vi "RUN regulateur MODBUS EPC3000.vi"(2 "Commentaires":string, 3 "Fichier rapport":path) -> (0 "error out":errorcluster caption="entrée d'erreur (pas d'erreur)", 1 "annulé":bool)   [LabVIEW 2022 SP3]
uses:
  Enum/Enum r5.ctl
  Variables globales/Variables glob EUROTHERM.vi
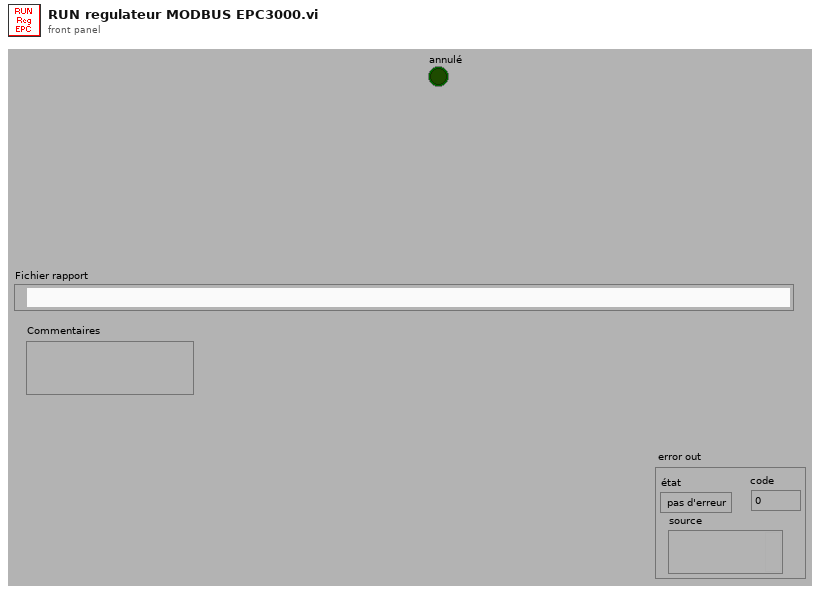
[diagram p1: front panel]
types:
  T1 = typedef "Enum r5.ctl" = enum16{"déja en run", "mesure hors gamme", "fichier rapport", "envoi run", "fin"}
  T2 = cluster{"Noms voies select acqui 1COM":string[]}[]
  T3 = typedef "Semaphore RefNum" = refnum<k1>
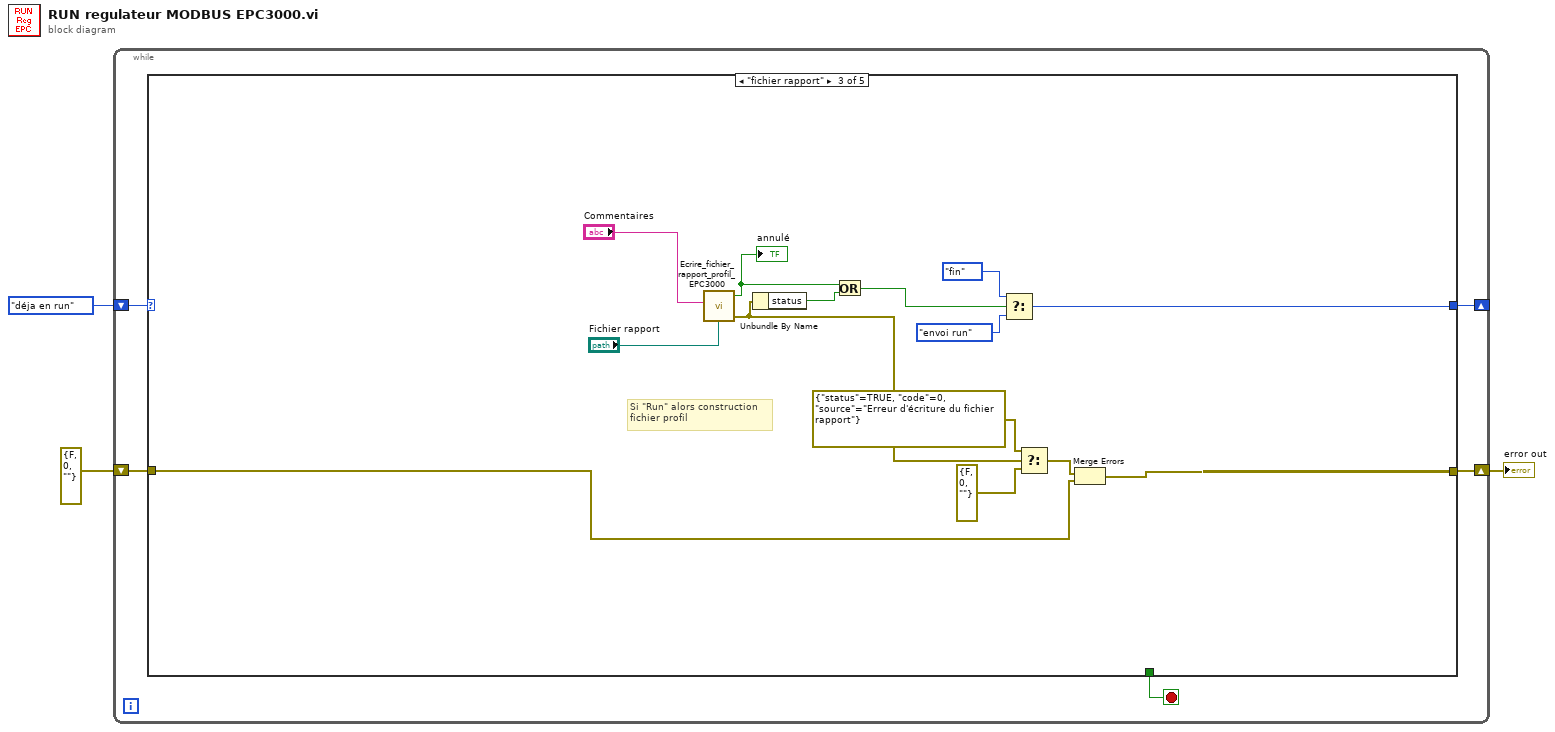
[diagram p0: block diagram]
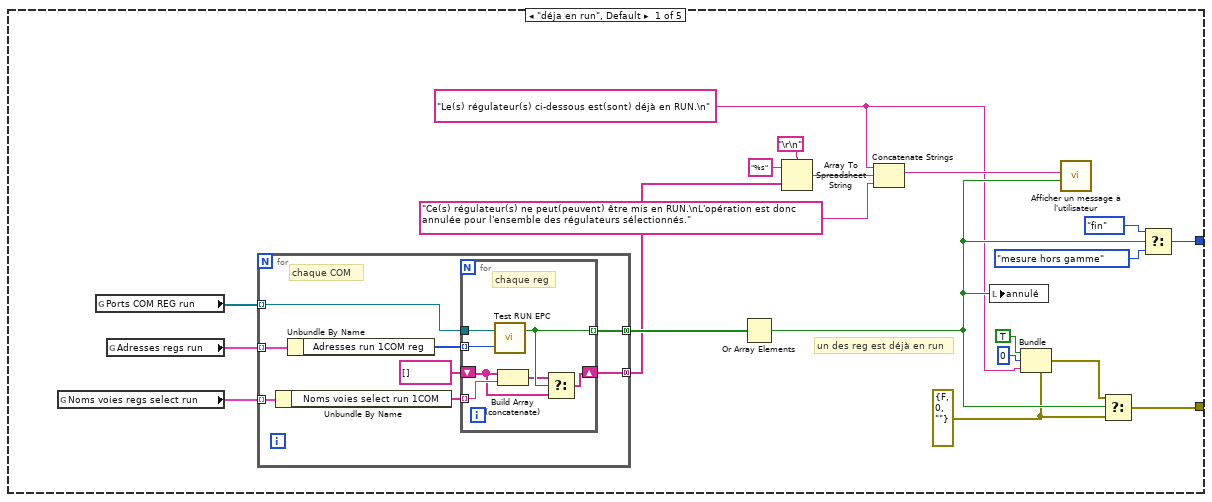
[diagram p2: hidden frame]
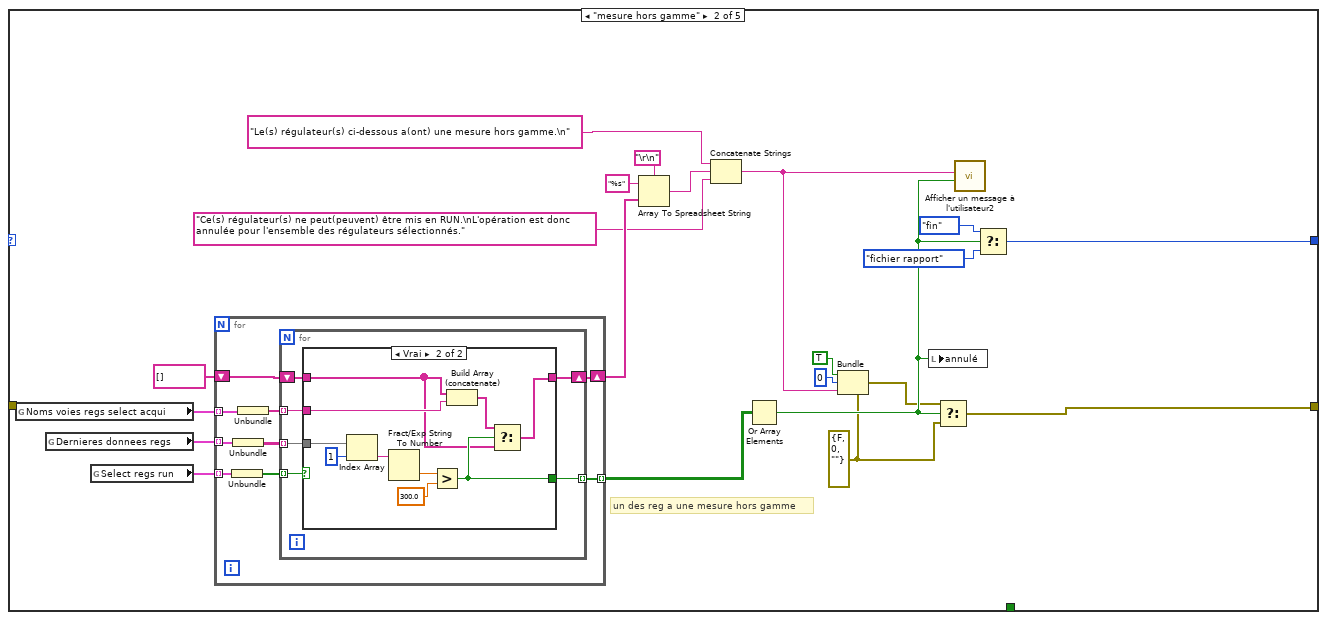
[diagram p3: hidden frame]
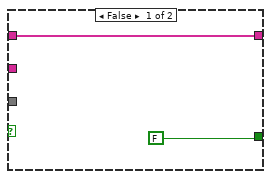
[diagram p4: hidden frame]
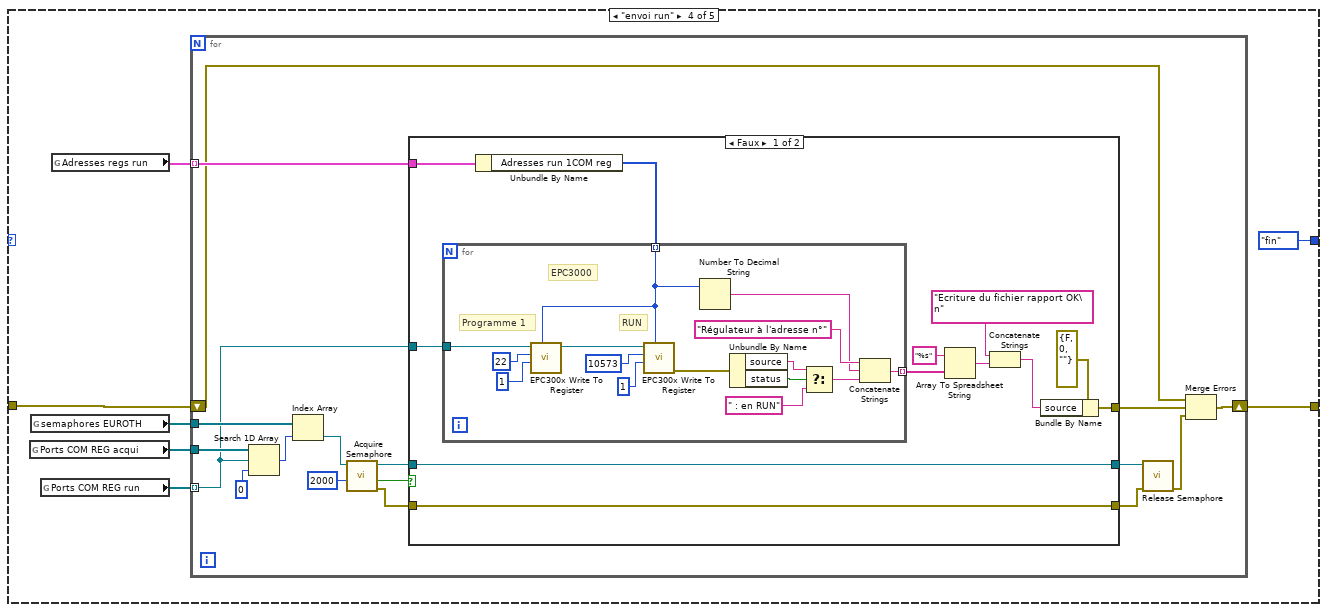
[diagram p5: hidden frame]
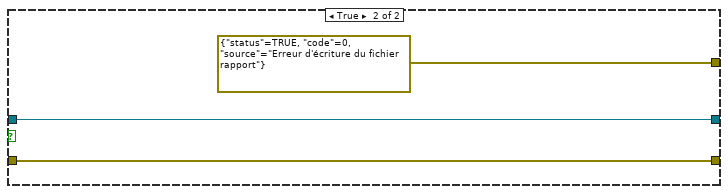
[diagram p6: hidden frame]
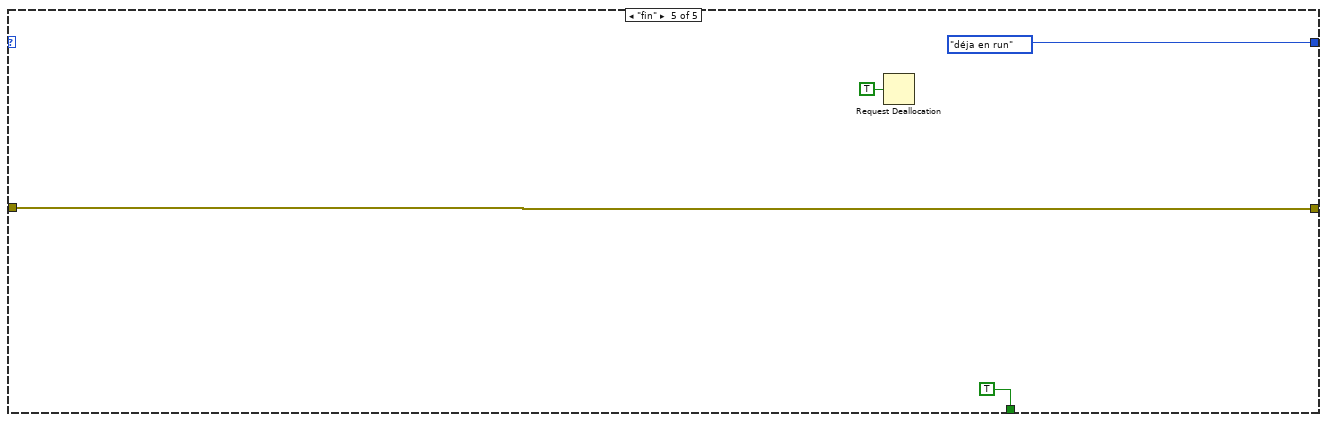
[diagram p7: hidden frame]
diagram:
  n1 = while {
    shift-right: [w6] -> _
    shift-left: Enum_r5."déja en run" ("Énum") -> [w8]
    shift-right: [w4] -> w1
    shift-left: errorcluster {"status"=FALSE, "code"=0, "source"=""} ("error fichier") -> [w5]
    stop <- w7 stop-if-true
    n2 = case shown="\"fichier rapport\"" w8 {
      tunnel: [_ _ _ _ TRUE] -> w7
      tunnel: [w25 w62 w101 Enum_r5."fin" ("Énum") Enum_r5."déja en run" ("Énum")] -> w6
      tunnel: w5 -> [_ _ w97 w108 w161]
      tunnel: [w24 w61 w96 w112 w161] -> w4
      frame "déja en run", Default {
        w12 = "Le(s) régulateur(s) ci-dessous est(sont) déjà en RUN.\n"
        w13 = errorcluster {"status"=FALSE, "code"=0, "source"=""} ("error fichier")
        # "un des reg est déjà en run"
        n3 = global read "Variables glob EUROTHERM.vi" "Noms voies regs select run"() -> (w21:cluster{"Noms voies select run 1COM":string[]}[])
        n4 = global read "Variables glob EUROTHERM.vi" "Ports COM REG run"() -> (w22:refnum<visa-resource-name>[])
        n5 = global read "Variables glob EUROTHERM.vi" "Adresses regs run"() -> (w23:cluster{"Adresses run 1COM reg":u16[]}[])
        n6 = for {
          tunnel: [w36] -> w28 mode=concatenating
          tunnel: w23 -> [w35] mode=indexing
          tunnel: w22 -> [w33] mode=indexing
          tunnel: w21 -> [w32] mode=indexing
          tunnel: [w30] -> w20 mode=concatenating
          # "chaque COM"
          n7 = Unbundle By Name(w32) -> ("Noms voies select run 1COM"=w31:string[])
          n8 = Unbundle By Name(w35) -> ("Adresses run 1COM reg"=w34:u16[])
          n9 = for {
            tunnel: w34 -> [w43] mode=indexing
            tunnel: [w41] -> w36 mode=indexing
            tunnel: w33 -> [w42]
            tunnel: w31 -> [w40] mode=indexing
            shift-right: [w38] -> w30
            shift-left: string[] [] -> [w37]
            # "chaque reg"
            n10 = call "Test RUN EPC.vi"("Adresse régulateur"=w43, "Port COM run 1 REG"=w42) -> ("En RUN"=w41:bool)  [unwired: 1 out]
            n11 = Build Array (concatenate)(w37, w40) -> (w39:string[])
            n12 = Select(t=w39, s=w41, f=w37) -> (s? t:f=w38:string[])
          }
        }
        n13 = Or Array Elements(Boolean array=w28) -> (logical OR=w17:bool)
        n14 = Array To Spreadsheet String(delimiter (Tab)="\r\n", array=w20, 3:"%s" ("chaîne de format")) -> (spreadsheet string=w19:string)
        n15 = Concatenate Strings(w12, w19, "Ce(s) régulateur(s) ne peut(peuvent) être mis en RUN.\nL'opération est donc annulée pour l'ensemble des régulateurs sélectionnés.") -> (w16:string)
        n16 = local write "annulé"(w17) -> ()
        n17 = Bundle(cluster=w13, "status"=TRUE, "code"=0, "source"=w12) -> (w11:errorcluster)
        n18 = call "Afficher un message à l'utilisateur"("Enable"=w17, "Message"=w16) -> ()  [unwired: 8 in, 2 out]
        n19 = Select(t=w11, s=w17, f=w13) -> (s? t:f=w24:errorcluster)
        n20 = Select(t=Enum_r5."fin" ("Énum"), s=w17, f=Enum_r5."mesure hors gamme" ("Énum")) -> (s? t:f=w25:T1)
      }
      frame "mesure hors gamme" {
        w56 = errorcluster {"status"=FALSE, "code"=0, "source"=""} ("error fichier")
        # "un des reg a une mesure hors gamme"
        n21 = global read "Variables glob EUROTHERM.vi" "Noms voies regs select acqui"() -> (w51:T2)
        n22 = global read "Variables glob EUROTHERM.vi" "Dernieres donnees regs"() -> (w59:cluster{"Dernieres donnees 1COM":string[][]}[])
        n23 = global read "Variables glob EUROTHERM.vi" "Select regs run"() -> (w58:cluster{"Sélect run 1COM reg":bool[]}[])
        n24 = for {
          tunnel: w59 -> [w73] mode=indexing
          tunnel: w58 -> [w71] mode=indexing
          tunnel: [w70] -> w57 mode=indexing
          tunnel: w51 -> [w68] mode=indexing
          shift-right: [w65] -> w48
          shift-left: string[] [] -> [w66]
          n25 = Unbundle(w71) -> ("Sélect run 1COM reg"=w69:bool[])
          n26 = Unbundle(w73) -> ("Dernieres donnees 1COM"=w72:string[][])
          n27 = Unbundle(w68) -> ("Noms voies select acqui 1COM"=w67:string[])
          n28 = for {
            tunnel: w72 -> [w79] mode=indexing
            tunnel: [w78] -> w70 mode=indexing
            tunnel: w69 -> [w77] mode=indexing
            tunnel: w67 -> [w76] mode=indexing
            shift-right: [w74] -> w65
            shift-left: w66 -> [w75]
            n29 = case shown="Vrai" w77 {
              tunnel: w79 -> [_ w90]
              tunnel: [FALSE w86] -> w78
              tunnel: w76 -> [_ w85]
              tunnel: w75 -> [w80 w83]
              tunnel: [w80 w82] -> w74
              frame False {
              }
              frame True {
                n30 = Index Array(array=w90, index=1 ("indice")) -> (element=w89:string)
                n31 = Fract/Exp String To Number(string=w89) -> (number=w88:dbl)  [unwired: 3 in, 1 out]
                n32 = Greater?(x=w88, y=300.0) -> (0:w86:bool)
                n33 = Build Array (concatenate)(w83, w85) -> (w84:string[])
                n34 = Select(t=w84, s=w86, f=w83) -> (s? t:f=w82:string[])
              }
            }
          }
        }
        n35 = Array To Spreadsheet String(delimiter (Tab)="\r\n", array=w48, 3:"%s" ("chaîne de format")) -> (spreadsheet string=w47:string)
        n36 = Concatenate Strings("Le(s) régulateur(s) ci-dessous a(ont) une mesure hors gamme.\n", w47, "Ce(s) régulateur(s) ne peut(peuvent) être mis en RUN.\nL'opération est donc annulée pour l'ensemble des régulateurs sélectionnés.") -> (w44:string)
        n37 = Or Array Elements(Boolean array=w57) -> (logical OR=w60:bool)
        n38 = Bundle(cluster=w56, "status"=TRUE, "code"=0, "source"=w44) -> (w52:errorcluster)
        n39 = local write "annulé"(w60) -> ()
        n40 = Select(t=w52, s=w60, f=w56) -> (s? t:f=w61:errorcluster)
        n41 = call "Afficher un message à l'utilisateur2"("Enable"=w60, "Message"=w44) -> ()  [unwired: 8 in, 2 out]
        n42 = Select(t=Enum_r5."fin" ("Énum"), s=w60, f=Enum_r5."fichier rapport" ("Énum")) -> (s? t:f=w62:T1)
      }
      frame "fichier rapport" {
        # "Si \"Run\" alors construction\nfichier profil"
        n43 = call "Ecrire_fichier_rapport_profil_EPC3000.vi"("Commentaires"="Commentaires", "Chemin du fichier rapport"="Fichier rapport") -> ("annulé"=w93:bool, "error out"=w95:errorcluster)  [unwired: 4 in]
        "annulé" <- w93
        n44 = Unbundle By Name(w95) -> ("status"=w94:bool)
        n45 = Or(x=w93, y=w94) -> (x .or. y?=w92:bool)
        n46 = Select(t=Enum_r5."fin" ("Énum"), s=w92, f=Enum_r5."envoi run" ("Énum")) -> (s? t:f=w101:T1)
        n47 = Select(t=errorcluster {"status"=TRUE, "code"=0, "source"="Erreur d'écriture du fichier rapport"} ("error fichier"), s=w95, f=errorcluster {"status"=FALSE, "code"=0, "source"=""} ("error fichier")) -> (s? t:f=w98:errorcluster)
        n48 = Merge Errors(w98, w97) -> (w96:errorcluster)
      }
      frame "envoi run" {
        n49 = global read "Variables glob EUROTHERM.vi" "Ports COM REG acqui"() -> (w107:refnum<visa-resource-name>[])
        n50 = global read "Variables glob EUROTHERM.vi" "semaphores EUROTH"() -> (w109:T3[])
        n51 = global read "Variables glob EUROTHERM.vi" "Ports COM REG run"() -> (w106:refnum<visa-resource-name>[])
        n52 = global read "Variables glob EUROTHERM.vi" "Adresses regs run"() -> (w110:cluster{"Adresses run 1COM reg":u16[]}[])
        n53 = for {
          tunnel: w110 -> [w120] mode=indexing
          tunnel: w109 -> [w119]
          shift-right: [w121] -> w112
          shift-left: w108 -> [w117]
          tunnel: w107 -> [w116]
          tunnel: w106 -> [w113] mode=indexing
          n54 = Search 1D Array(1D array=w116, element=w113, start index (0)=0 ("indice de départ (0)")) -> (index of element=w114:i32)
          n55 = Index Array(array=w119, index=w114) -> (element=w118:T3)
          n56 = call <vilib>:"Acquire Semaphore.vi"("ms timeout (-1)"=2000, "semaphore"=w118) -> ("error out"=w124:errorcluster, "timed out"=w122:bool, "semaphore out"=w123:T3)  [unwired: 3 in]
          n57 = case shown="Faux" w122 {
            tunnel: w123 -> [w141 w159]
            tunnel: w124 -> [w140 w158]
            tunnel: [w141 w159] -> w126
            tunnel: [w140 w158] -> w127
            tunnel: [w139 errorcluster {"status"=TRUE, "code"=0, "source"="Erreur d'écriture du fichier rapport"} ("error fichier")] -> w128
            tunnel: w120 -> [w132 _]
            tunnel: w113 -> [w130 _]
            frame False {
              n58 = Unbundle By Name(w132) -> ("Adresses run 1COM reg"=w131:u16[])
              n59 = for {
                tunnel: w131 -> [w142] mode=indexing
                tunnel: [w152] -> w138 mode=indexing
                tunnel: w130 -> [w144]
                # "Programme 1"
                # "RUN"
                # "EPC3000"
                n60 = call "EPC300x Write To Register.vi"("Unit Address (1)"=w142, "Data (0)"=i16 1, "Register Address (0)"=22, "VISA session"=w144) -> ("dup VISA session"=w143:refnum<visa-resource-name>)  [unwired: 6 in, 1 out]
                n61 = call "EPC300x Write To Register.vi"("Unit Address (1)"=w142, "Data (0)"=i16 1, "Register Address (0)"=u16 10573, "VISA session"=w143) -> ("error out"=w149:errorcluster)  [unwired: 6 in, 1 out]
                n62 = Number To Decimal String(number=w142) -> (decimal integer string=w154:string)  [unwired: 1 in]
                n63 = Unbundle By Name(w149) -> ("source"=w150:string, "status"=w151:bool)
                n64 = Select(t=w150, s=w151, f=" : en RUN" ("chaîne")) -> (s? t:f=w153:string)
                n65 = Concatenate Strings("Régulateur à l'adresse n°", w154, w153) -> (w152:string)
              }
              n66 = Array To Spreadsheet String(array=w138, 3:"%s" ("chaîne de format")) -> (spreadsheet string=w135:string)  [unwired: 1 in]
              n67 = Concatenate Strings("Ecriture du fichier rapport OK\n" ("source"), w135) -> (w133:string)
              n68 = Bundle By Name(cluster=errorcluster {"status"=FALSE, "code"=0, "source"=""} ("error fichier"), "source"=w133) -> (w139:errorcluster)
            }
            frame True {
            }
          }
          n69 = call <vilib>:"Release Semaphore.vi"("error in (no error)"=w127, "semaphore"=w126) -> ("error out"=w129:errorcluster)  [unwired: 4 in, 1 out]
          n70 = Merge Errors(w117, w128, w129) -> (w121:errorcluster)
        }
      }
      frame "fin" {
        n71 = Request Deallocation(TRUE ("flag")) -> ()
      }
    }
  }
  "error out" <- w1
